vi "Kinect - Land (SubVI).vi"(8 "error in (no error)":errorcluster, 11 "Array of Joint Positions In":dbl[][](array[numeric])) -> (0 "error out":errorcluster, 2 "Toggle Land/Take off":bool, 3 "Array of Joint Positions Out":dbl[][](array[numeric]))   [LabVIEW 2014]
panel:
  in  "Maximal distance between hands":dbl=0.25
  out "Distance between hands":dbl(knob)=0.1448702604855027 scale=0.0..1.5
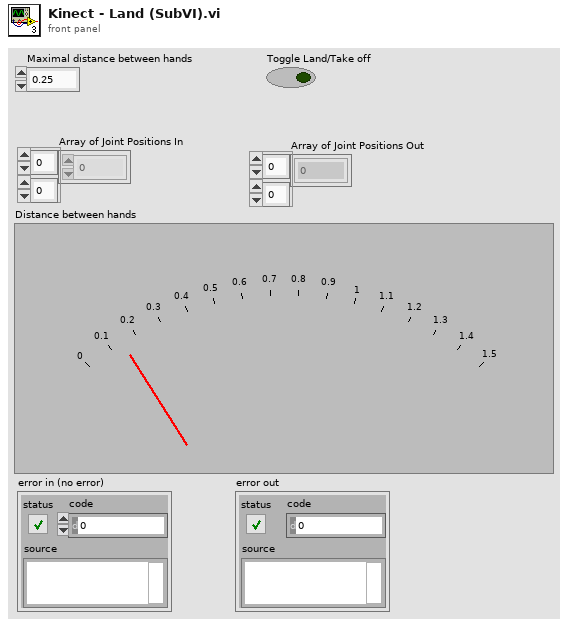
[diagram p1: front panel]
types:
  T1 = enum16{"hip centre", "spine", "shoulder centre", "head", "shoulder left", "elbow left", "wrist left", "hand left", "shoulder right", "elbow right", "wrist right", "hand right", "hip left", "knee left", "ankle left", "foot left", "hip right", "knee right", "ankle right", "foot right"}
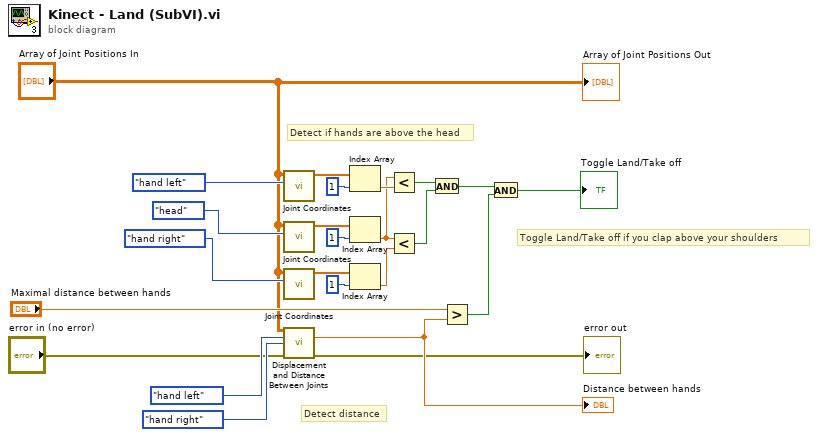
[diagram p0: block diagram]
diagram:
  # "Toggle Land/Take off if you clap above your shoulders"
  # "Detect if hands are above the head"
  # "Detect distance"
  n1 = call <vilib>:"Joint Coordinates.vi"("Joint 1"=T1."hand left", "Array of Joint Positions"="Array of Joint Positions In") -> ("Joint Coordinates"=w16:dbl[])  [unwired: 8 in, 1 out]
  n2 = call <vilib>:"Joint Coordinates.vi"("Joint 1"=T1."head", "Array of Joint Positions"="Array of Joint Positions In") -> ("Joint Coordinates"=w7:dbl[])  [unwired: 8 in, 1 out]
  n3 = call <vilib>:"Joint Coordinates.vi"("Joint 1"=T1."hand right", "Array of Joint Positions"="Array of Joint Positions In") -> ("Joint Coordinates"=w12:dbl[])  [unwired: 8 in, 1 out]
  n4 = call <vilib>:"Displacement and Distance Between Joints.vi"("Array of Joint Positions"="Array of Joint Positions In", "Joint 1"=T1."hand left", "Joint 2"=T1."hand right", "error in (no error)"="error in (no error)") -> ("Absolute Distance Between Joints"=w23:dbl, "error out"=→"error out":errorcluster)  [unwired: 9 in, 1 out]
  "Distance between hands" <- w23
  n5 = Index Array(array=w16, index=1) -> (element=w15:dbl)
  n6 = Index Array(array=w7, index=1) -> (element=w6:dbl)
  n7 = Index Array(array=w12, index=1) -> (element=w11:dbl)
  n8 = Less?(x=w6, y=w15) -> (x < y?=w5:bool)
  n9 = Less?(x=w6, y=w11) -> (x < y?=w4:bool)
  n10 = And(x=w5, y=w4) -> (x .and. y?=w2:bool)
  n11 = Greater?(x="Maximal distance between hands", y=w23) -> (0:w1:bool)
  n12 = And(x=w2, y=w1) -> (x .and. y?=→"Toggle Land/Take off":bool)
  "Array of Joint Positions Out" <- "Array of Joint Positions In"
